vi "Set Connector Pane Pattern.vi"(0 "Connector Pane":refnum<vi>, 1 "Pattern":u16(ring) items=["4800", "4801", "4802", "4803", "4804", "4805", "4806", "4807", "4808", "4809", "4810", "4811", "4812", "4813", "4814", "4815", "4816", "4817", "4818", "4819", "4820", "4821", "4822", "4823", "4824", "4825", "4826", "4827", "4828", "4829", "4830", "4831", "4832", "4833", "4834", "4835"], 2 "Flip Horizontal":bool, 3 "Flip Vertical":bool, 4 "Rotate 90 Deg.":bool, 5 "error in (no error)":errorcluster) -> (6 "Connector Pane Out":refnum<vi>, 7 "Number of Terminals":i32, 8 "error out":errorcluster)   [LabVIEW 2012, in "Scripting Tools.lvlib"]
doc: "Sets the connector pane pattern"
uses:
  Scripting Tools.lvlib
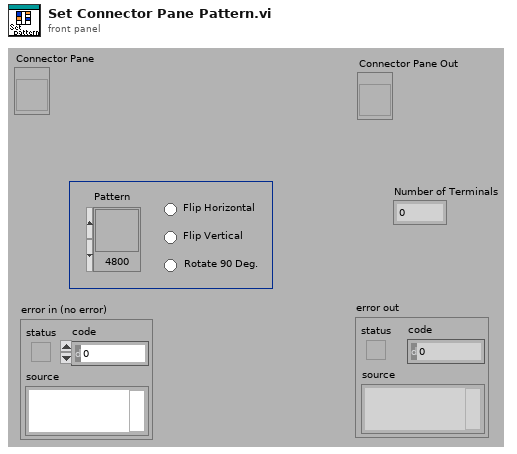
[diagram p1: front panel]
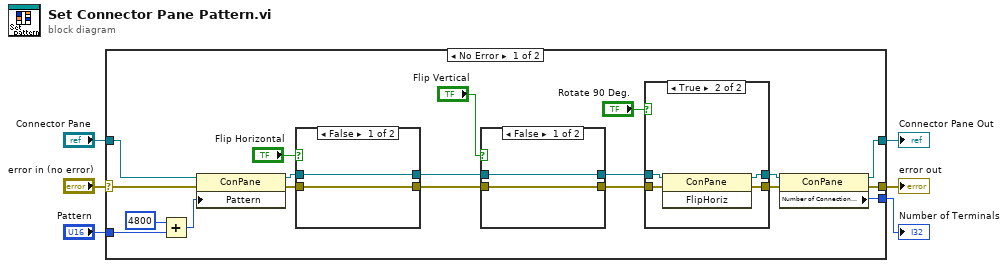
[diagram p0: block diagram]
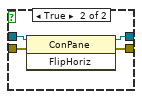
[diagram p3: hidden frame]
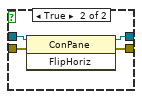
[diagram p4: hidden frame]
diagram:
  n1 = case shown="No Error" "error in (no error)" {
    selector: "error in (no error)" -> [w9 w45]
    tunnel: "Pattern" -> [w7 _]
    tunnel: "Connector Pane" -> [w25 w44]
    tunnel: [w12 w44] -> w4
    tunnel: [w11 _] -> w3
    tunnel: [w10 w45] -> w2
    frame No Error {
      n2 = Add(x=u16 4800 ("y"), y=w7) -> (x+y=w8:u16)
      n3 = property on="Property Node" class="ConPane"(reference=w25, error in=w9, "Pattern"=w8) -> (reference out=w23:refnum<vi>, error out=w22:errorcluster)
      n4 = case shown="False" "Flip Horizontal" {
        tunnel: w23 -> [w39 w43]
        tunnel: w22 -> [w38 w42]
        tunnel: [w39 w41] -> w21
        tunnel: [w38 w40] -> w20
        frame False {
        }
        frame True {
          n5 = invoke on="Invoke Node" class="ConPane" method="FlipHoriz"(reference=w43, error in=w42) -> (reference out=w41:refnum<vi>, error out=w40:errorcluster)  [unwired: 1 in, 1 out]
        }
      }
      n6 = case shown="False" "Flip Vertical" {
        tunnel: w21 -> [w33 w37]
        tunnel: w20 -> [w32 w36]
        tunnel: [w33 w35] -> w19
        tunnel: [w32 w34] -> w18
        frame False {
        }
        frame True {
          n7 = invoke on="Invoke Node" class="ConPane" method="FlipHoriz"(reference=w37, error in=w36) -> (reference out=w35:refnum<vi>, error out=w34:errorcluster)  [unwired: 1 in, 1 out]
        }
      }
      n8 = case shown="True" "Rotate 90 Deg." {
        tunnel: w19 -> [w27 w31]
        tunnel: w18 -> [w26 w30]
        tunnel: [w27 w29] -> w13
        tunnel: [w26 w28] -> w14
        frame False {
        }
        frame True {
          n9 = invoke on="Invoke Node" class="ConPane" method="FlipHoriz"(reference=w31, error in=w30) -> (reference out=w29:refnum<vi>, error out=w28:errorcluster)  [unwired: 1 in, 1 out]
        }
      }
      n10 = property on="Property Node" class="ConPane"(reference=w13, error in=w14) -> (reference out=w12:refnum<vi>, error out=w10:errorcluster, "Number of Connection Terminals"=w11:u32)
    }
    frame Error {
    }
  }
  "Connector Pane Out" <- w4
  "error out" <- w2
  "Number of Terminals" <- w3
